vi "LocalizedStrings.vi"() -> ()   [LabVIEW 2023, in "GettingStartedWindow.lvlib"]
uses:
  <resource>/modes/FRC/GettingStartedWindow.lvlib
panel:
  in  "TargetDevices_button_CH":string
  in  "TargetDevices_CH":string
  in  "Search_CH":string
  in  "Search_Help_button_CH":string
  in  "Search_Help_CH":string
  in  "Close":string
  in  "PDF_failure_message":string
  in  "TargetButtonBooleanText":string
  in  "GettingStarted":string
  in  "NISearchHint":string
  in  "LVState_Unknown":string
  in  "LVState_DebugDeployment":string
  in  "LVState_Player":string
  in  "LVState_Student":string
  in  "LVState_Eval":string
  in  "LVState_Pro":string
  in  "LVState_Full":string
  in  "LVState_Base":string
  in  "LVState_Failure":string
  in  "NonWindowsLabVIEWInfoMessage":string
  in  "SearchButtonBooleanText":string
  in  "SearchHelpLabel":string
  in  "ResourcesColumnHeader":string
  in  "FilesColumnHeader":string
  # "Used in GWS_LabVIEWState.vi"
  # "These globals are populated\nfrom the XML file."
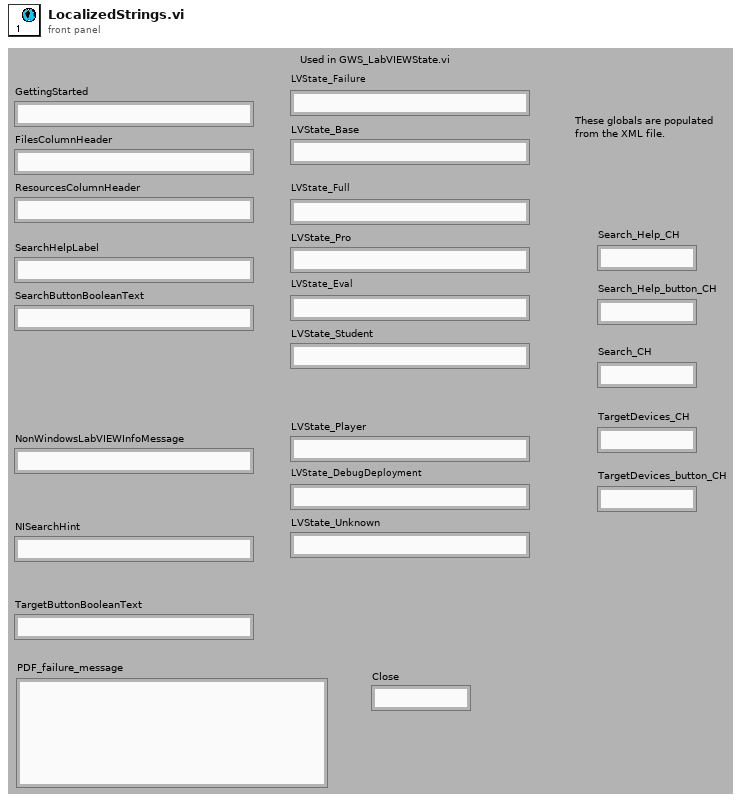
[diagram p1: front panel]
diagram:
